vi "OT Spectra to FlexLogger.vi"(4 "Timing Reference":waveform(dbl), 5 "Settings":T1={"channels"=1, "orders"=[1.0, 2.0, 24.0], "band half-width (orders)"=0.2, "window ENBW (bins)"=1.5}, 6 "reset? (F)":bool, 7 "magnitude":dbl[][](array[numeric]), 8 "error in (no error)":errorcluster, 9 "delta order":dbl[](array[numeric]), 10 "order 0":dbl[](array[numeric]), 11 "speed [RPM]":dbl[](array[numeric])) -> (0 "error out":errorcluster, 2 "Values":dbl[](array[numeric]), 3 "Array of Waveforms":waveform(dbl)[](array[waveform]))   [LabVIEW 2026]
doc: "Turns the outputs of the order power spectrum example into FlexLogger channels: RPM plus one order amplitude (EU rms) per accel channel and per order.\n\nInputs come straight from the example diagram:\n- speed [RPM]: the speed profile speed array of this block (OAT Analog Tacho Process). RPM = its last point.\n- order 0 / delta order / magnitude: the order power spectra unbundled in a For Loop (one element or row per accel channel). magnitude must be LINEAR power (dB on? = FALSE on OAT Order Power Spectrum).\n\nOrder amplitude = sqrt( sum of the magnitude bins within order +/- band half-width / window ENBW ). ENBW = 1.5 for Hanning. This is the same math as SVFA Power in Band.\n\nOutput Array of Waveforms (to Write 1D Wfm with Auto Calculate T0 = TRUE): one 1-point waveform per channel with t0 = block t0 and dt = block length, in this order:\nRPM, then for accel channel 0 one amplitude per order, then channel 1, and so on.\nInitialize must create the same channels in the same order: 1 + channels x orders.\n\nNo new tach edges or no new spectrum in a block (empty arrays) -> the last values are repeated (the While Loop shift register keeps them between calls, so this VI must stay preallocated reentrant). Every channel is written every block. Before the first result the values are 0.\nchannels in Settings must equal the number of accel channels in the spectra.\nreset? TRUE on the first Process call after Configure Session."
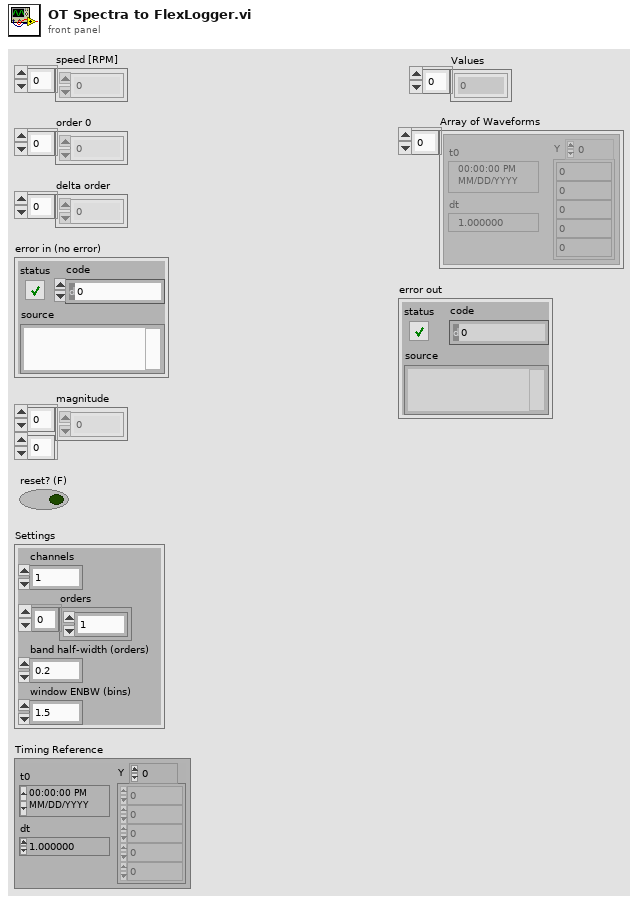
[diagram p1: front panel]
types:
  T1 = cluster{"channels":i32, "orders":dbl[], "band half-width (orders)":dbl, "window ENBW (bins)":dbl}
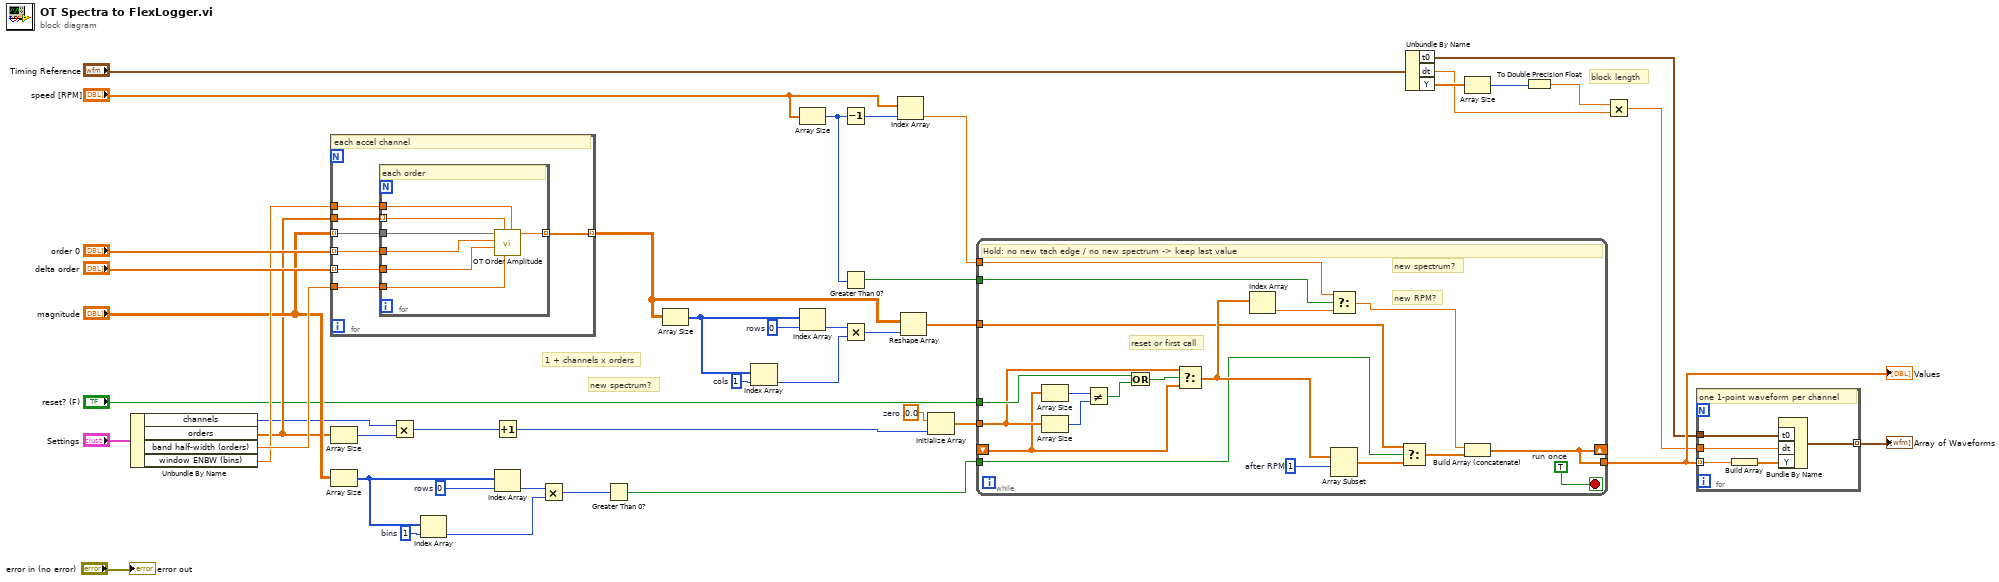
[diagram p0: block diagram]
diagram:
  w18 = 0.0  # zero
  w26 = 1  # bins
  w28 = 0  # rows
  w34 = 1  # cols
  w36 = 0  # rows
  # "block length"
  # "1 + channels x orders"
  # "new spectrum?"
  n1 = Unbundle By Name("Settings") -> ("channels"=w21:i32, "orders"=w22:dbl[], "band half-width (orders)"=w38:dbl, "window ENBW (bins)"=w37:dbl)
  n2 = for {
    tunnel: "magnitude" -> [w50] mode=indexing
    tunnel: "order 0" -> [w49] mode=indexing
    tunnel: "delta order" -> [w48] mode=indexing
    tunnel: w22 -> [w51]
    tunnel: w38 -> [w47]
    tunnel: w37 -> [w46]
    tunnel: [w45] -> w31 mode=indexing
    # "each accel channel"
    n3 = for {
      tunnel: w51 -> [w55] mode=indexing
      tunnel: w50 -> [w58]
      tunnel: w49 -> [w57]
      tunnel: w48 -> [w56]
      tunnel: w47 -> [w54]
      tunnel: w46 -> [w53]
      tunnel: [w52] -> w45 mode=indexing
      # "each order"
      n4 = call "OT Order Amplitude.vi"("window ENBW (bins)"=w53, "band half-width (orders)"=w54, "order"=w55, "delta order"=w56, "order 0"=w57, "magnitude"=w58) -> ("amplitude (EU rms)"=w52:dbl)  [unwired: 5 in]
    }
  }
  n5 = Array Size(array=w22) -> (size(s)=w20:i32)
  n6 = Array Size(array="magnitude") -> (size(s)=w27:i32[])
  n7 = Multiply(x=w21, y=w20) -> (x*y=w19:i32)
  n8 = Index Array(array=w27, index=w26) -> (element=w24:i32)
  n9 = Increment(x=w19) -> (x+1=w17:i32)
  n10 = Index Array(array=w27, index=w28) -> (element=w25:i32)
  n11 = Multiply(x=w25, y=w24) -> (x*y=w23:i32)
  n12 = Greater Than 0?(x=w23) -> (x > 0?=w12:bool)
  n13 = Array Size(array=w31) -> (size(s)=w35:i32[])
  n14 = Index Array(array=w35, index=w34) -> (element=w32:i32)
  n15 = Array Size(array="speed [RPM]") -> (size(s)=w43:i32)
  n16 = Index Array(array=w35, index=w36) -> (element=w33:i32)
  n17 = Decrement(x=w43) -> (x-1=w41:i32)
  n18 = Greater Than 0?(x=w43) -> (x > 0?=w14:bool)
  n19 = Multiply(x=w33, y=w32) -> (x*y=w30:i32)
  n20 = Index Array(array="speed [RPM]", index=w41) -> (element=w13:dbl)
  n21 = Reshape Array(w31, w30) -> (w11:dbl[])
  n22 = Initialize Array(w18, w17) -> (w16:dbl[])
  n23 = while {
    tunnel: w16 -> [w73]
    tunnel: "reset? (F)" -> [w75]
    tunnel: w14 -> [w67]
    tunnel: w13 -> [w68]
    tunnel: w12 -> [w64]
    tunnel: w11 -> [w65]
    shift-right: [w59] -> _
    shift-left: _ -> [w71]
    tunnel: [w59] -> w5
    stop <- w60 stop-if-true
    w60 = TRUE  # run once
    w69 = 1  # after RPM
    # "new spectrum?"
    # "new RPM?"
    # "reset or first call"
    # "Hold: no new tach edge / no new spectrum -> keep last value"
    n24 = Array Size(array=w71) -> (size(s)=w77:i32)
    n25 = Array Size(array=w73) -> (size(s)=w76:i32)
    n26 = Not Equal?(x=w77, y=w76) -> (x != y?=w74:bool)
    n27 = Or(x=w75, y=w74) -> (x .or. y?=w72:bool)
    n28 = Select(t=w73, s=w72, f=w71) -> (s? t:f=w70:dbl[])
    n29 = Index Array(array=w70) -> (element=w66:dbl)  [unwired: 1 in]
    n30 = Select(t=w68, s=w67, f=w66) -> (s? t:f=w62:dbl)
    n31 = Array Subset(array=w70, index=w69) -> (w63:dbl[])  [unwired: 1 in]
    n32 = Select(t=w65, s=w64, f=w63) -> (s? t:f=w61:dbl[])
    n33 = Build Array (concatenate)(w62, w61) -> (w59:dbl[])
  }
  "Values" <- w5
  n34 = Unbundle By Name("Timing Reference") -> ("t0"=w4:timestamp, "dt"=w6:dbl, "Y"=w9:dbl[])
  n35 = Array Size(array=w9) -> (size(s)=w8:i32)
  n36 = To Double Precision Float(number=w8) -> (double precision float=w7:dbl)
  n37 = Multiply(x=w7, y=w6) -> (x*y=w3:dbl)
  n38 = for {
    tunnel: w5 -> [w82] mode=indexing
    tunnel: w4 -> [w81]
    tunnel: w3 -> [w80]
    tunnel: [w78] -> w2 mode=indexing
    # "one 1-point waveform per channel"
    n39 = Build Array(w82) -> (w79:dbl[])
    n40 = Bundle By Name("t0"=w81, "dt"=w80, "Y"=w79) -> (w78:waveform(dbl))  [unwired: 1 in]
  }
  "Array of Waveforms" <- w2
  "error out" <- "error in (no error)"
